vi "Write Tags.vi"() -> ()   [LabVIEW 2018, in "Library.lvlib"]
uses:
  Library.lvlib
  <vilib>/Skyline/Tag/Shared/typedefs/DataType.ctl
  <vilib>/Skyline/Tag/Wrapper/Wrapper_class/Generate Tag Cluster (DBL) 2.vi
  <vilib>/Skyline/Tag/Shared/Serialize Double to String.vi
  <vilib>/Skyline/Tag/Wrapper/Wrapper HTTP_class/Open Tag HTTP.vi
  <vilib>/Skyline/Tag/Wrapper/Wrapper_class/Generate Tag Cluster Core 2.vi
  <vilib>/Skyline/Tag/Wrapper/Wrapper_class/Close Tag (Multiple).vi
  <vilib>/Skyline/Configuration/Configuration_class/NI Skyline Configuration.lvclass
  <vilib>/Skyline/Tag/Wrapper/Wrapper_class/NI Skyline Tag.lvclass
  <vilib>/Skyline/Tag/Shared/NI Skyline Tag.lvlib
  <vilib>/Skyline/Configuration/Configuration HTTP_class/NI Skyline Configuration HTTP.lvclass
  <vilib>/Skyline/Configuration/Configuration HTTP_class/Open Configuration HTTP.vi
  <vilib>/Skyline/Configuration/Configuration AMQP_class/Open Configuration AMQP.vi
  <vilib>/Skyline/Configuration/Configuration AMQP_class/NI Skyline Configuration AMQP.lvclass
  <vilib>/Skyline/Tag/Wrapper/Wrapper HTTP_class/NI Skyline Tag HTTP.lvclass
panel:
  in  "Stop":bool
  out "Inner Temp":dbl(graph) caption="Inner Temp (F)"
  out "Outer Temp":dbl(graph) caption="Outer Temp (F)"
  # "Overview: Demonstrates the use of the SystemLink Tag API to write multiple tag values. Use tags to publish and monitor live measurement data.\n\nRequirements: G Web Development Software\n\nInstructions:\n1. Ensure the local SystemLink Server is running or you have access to SystemLink Cloud\n2. Determine if this example is connecting to data available on SystemLink Server or SystemLink Cloud and use the appropriate version of Open Configuration.vi \n3. Run this VI\n4. Monitor data published by this VI by running either Basic Data Services > Read Tags.gviweb or Full Data Services App > index.gviweb in webvi-examples\\CallSystemLinkDataServices\\Call SystemLink Data Services.gwebproject"
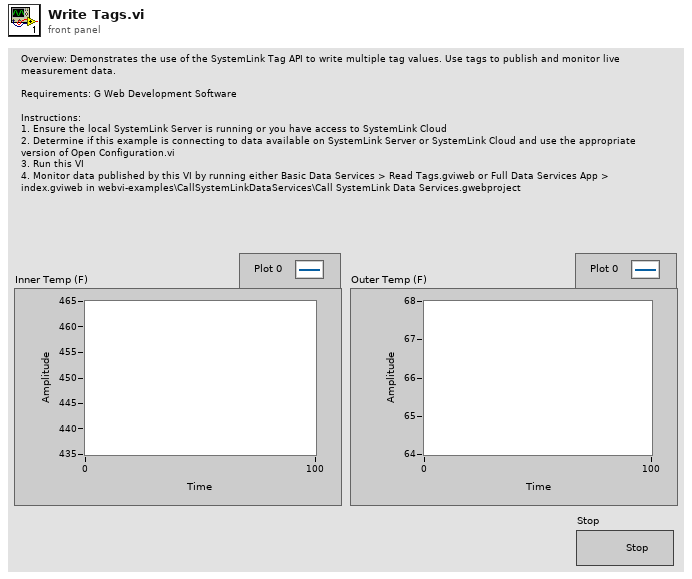
[diagram p1: front panel]
types:
  T1 = typedef "NI Skyline Tag.lvlib/DataType.ctl" = enum32{"Double", "I32", "String", "Boolean", "U64", "Timestamp"}
  T2 = typedef "NI Skyline Tag.lvclass/Tag Value Cluster Wrapper.ctl" = cluster{"Configuration":refnum<class "NI Skyline Configuration.lvclass">, "Tag Cluster":T3}
  T3 = typedef "NI Skyline Tag.lvlib/Tag Value Cluster.ctl" = cluster{"Path":string, "Workspace ID":string, "Data Type":T1, "Value":string, "Time Stamp":timestamp}
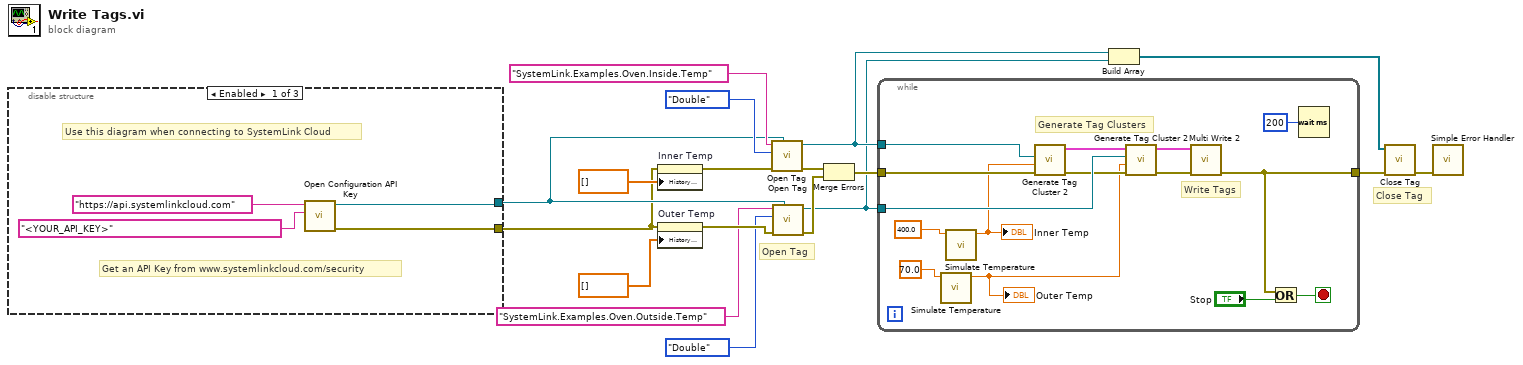
[diagram p0: block diagram]
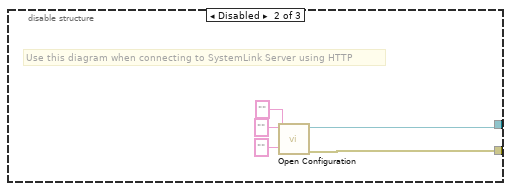
[diagram p2: hidden frame]
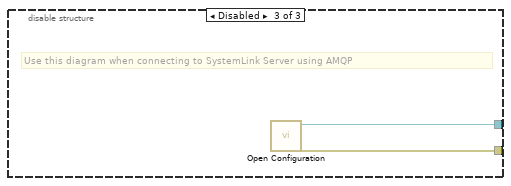
[diagram p3: hidden frame]
diagram:
  # "Close Tag"
  # "Open Tag"
  n1 = disable-structure shown="Enabled" {
    disable-tunnel: [w22 w23 w29] -> w2
    disable-tunnel: [w21 w27 w28] -> w1
    frame Enabled {
      # "Get an API Key from www.systemlinkcloud.com/security"
      # "Use this diagram when connecting to SystemLink Cloud"
      n2 = call <vilib>:"Open Configuration API Key.vi"("api key"="<YOUR_API_KEY>", "server url"="https://api.systemlinkcloud.com") -> ("error out"=w21:errorcluster, "configuration"=w22:refnum<class "NI Skyline Configuration HTTP.lvclass">)  [unwired: 8 in]
    }
    frame Disabled {
      # "Use this diagram when connecting to SystemLink Server using HTTP"
      n3 = call-poly <vilib>:"Open Configuration.vi"("password"="", "username"="", "server url"="") -> ("error out"=w27:errorcluster, "configuration"=w23:refnum<class "NI Skyline Configuration HTTP.lvclass">)  [unwired: 7 in]
    }
    frame Disabled {
      # "Use this diagram when connecting to SystemLink Server using AMQP"
      n4 = call-poly <vilib>:"Open Configuration.vi"() -> ("error out"=w28:errorcluster, "configuration"=w29:refnum<class "NI Skyline Configuration AMQP.lvclass">)  [unwired: 10 in]
    }
  }
  n5 = property on="Inner Temp" class="WFChart (strict)"(error in=w1, "History Data"=dbl[] []) -> (error out=w13:errorcluster)  [unwired: 1 in, 1 out]
  n6 = property on="Outer Temp" class="WFChart (strict)"(error in=w1, "History Data"=dbl[] []) -> (error out=w14:errorcluster)  [unwired: 1 in, 1 out]
  n7 = call-poly <vilib>:"Open Tag.vi"("configuration"=w2, "error in (no error)"=w13, "Data Type"=DataType."Double", "path"="SystemLink.Examples.Oven.Inside.Temp" ("tag path")) -> ("error out"=w18:errorcluster, "tag"=w5:refnum<class "NI Skyline Tag.lvclass">)  [unwired: 6 in]
  n8 = call-poly <vilib>:"Open Tag.vi"("configuration"=w2, "error in (no error)"=w14, "Data Type"=DataType."Double", "path"="SystemLink.Examples.Oven.Outside.Temp" ("tag path")) -> ("error out"=w17:errorcluster, "tag"=w3:refnum<class "NI Skyline Tag.lvclass">)  [unwired: 6 in]
  n9 = Merge Errors(w18, w17) -> (w16:errorcluster)
  n10 = while {
    tunnel: w5 -> [w40]
    tunnel: w3 -> [w39]
    tunnel: [w41] -> w11
    tunnel: w16 -> [w38]
    stop <- w42 stop-if-true
    # "Write Tags"
    # "Generate Tag Clusters"
    n11 = call "Simulate Temperature.vi"("Starting Temp"=70.0) -> ("Temp (F)"=w31:dbl)  [unwired: 10 in]
    "Outer Temp" <- w31
    n12 = call "Simulate Temperature.vi"("Starting Temp"=400.0) -> ("Temp (F)"=w30:dbl)  [unwired: 10 in]
    "Inner Temp" <- w30
    n13 = call-poly <vilib>:"Generate Tag Cluster 2.vi"("error in (no error)"=w38, "value"=w30, "tag in"=w40) -> ("error out"=w37:errorcluster, "tag clusters out"=w34:T2[])  [unwired: 6 in, 1 out]
    n14 = call-poly <vilib>:"Generate Tag Cluster 2.vi"("error in (no error)"=w37, "value"=w31, "tag in"=w39, "tag clusters in"=w34) -> ("error out"=w36:errorcluster, "tag clusters out"=w35:T2[])  [unwired: 5 in, 1 out]
    n15 = call <vilib>:"Multi Write 2.vi"("error in (no error)"=w36, "tag clusters"=w35) -> ("error out"=w41:errorcluster)  [unwired: 9 in]
    n16 = Or(x=w41, y="Stop") -> (x .or. y?=w42:bool)
    n17 = Wait (ms)(milliseconds to wait=u32 200) -> ()  [unwired: 1 out]
  }
  n18 = Build Array(w5, w3) -> (w4:refnum<class "NI Skyline Tag.lvclass">[])
  n19 = call-poly <vilib>:"Close Tag.vi"("error in (no error)"=w11, "tags"=w4) -> ("error out"=w10:errorcluster)  [unwired: 9 in]
  n20 = call <vilib>:"Simple Error Handler.vi"("error in (no error)"=w10) -> ()  [unwired: 4 in, 5 out]
